vi "Query Mast Position.vi"(8 "error in (no error)":errorcluster, 11 "CO3000 in":refnum<class "CO3000.lvclass">) -> (0 "error out":errorcluster, 2 "Current Position (in cm)":i32, 3 "CO3000 out":refnum<class "CO3000.lvclass">)   [LabVIEW 2023, in "Turn Table and Mast.lvlib" / "CO3000.lvclass"]
uses:
  CO3000.lvclass
  CO3000.lvclass/CO3000.ctl
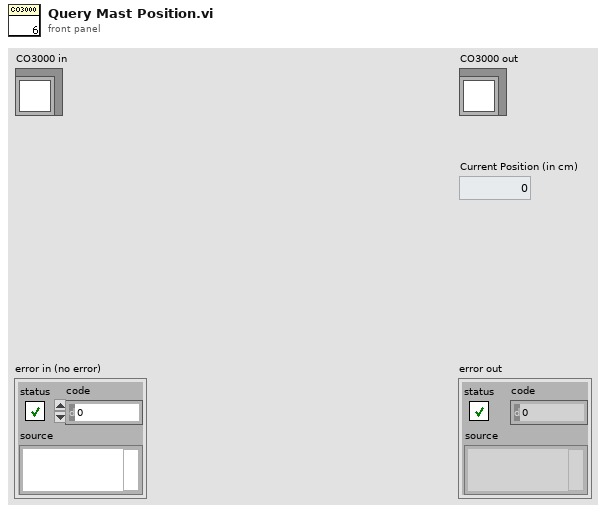
[diagram p1: front panel]
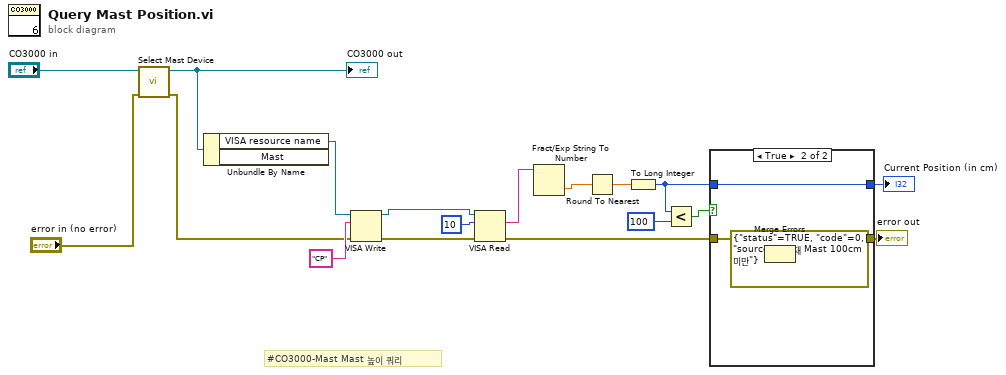
[diagram p0: block diagram]
diagram:
  # "#CO3000-Mast Mast 높이 쿼리"
  n1 = call "Select Mast Device.vi"("error in (no error)"="error in (no error)", "CO3000 in"="CO3000 in") -> ("error out"=w2:errorcluster, "CO3000 out"=w1:refnum<class "CO3000.lvclass">)  [unwired: 8 in]
  "CO3000 out" <- w1
  n2 = Unbundle By Name(w1) -> ("VISA resource name"=w14:refnum<visa-resource-name>)  [unwired: 1 out]
  n3 = VISA Write(VISA resource name=w14, write buffer="CP" ("버퍼 쓰기"), error in (no error)=w2) -> (VISA resource name out=w16:refnum<visa-resource-name>, error out=w17:errorcluster)  [unwired: 1 out]
  n4 = VISA Read(VISA resource name=w16, byte count=u32 10 ("바이트 카운트"), error in (no error)=w17) -> (read buffer=w13:string, error out=w6:errorcluster)  [unwired: 2 out]
  n5 = Fract/Exp String To Number(string=w13) -> (number=w12:dbl)  [unwired: 3 in, 1 out]
  n6 = Round To Nearest(number=w12) -> (nearest integer value=w11:dbl)
  n7 = To Long Integer(number=w11) -> (32bit integer=w8:i32)
  n8 = Less?(x=w8, y=100) -> (x < y?=w9:bool)
  n9 = case shown="True" w9 {
    tunnel: w8 -> [w20 w24]
    tunnel: [w20 w24] -> w7
    tunnel: w6 -> [w19 w22]
    tunnel: [w19 w21] -> w5
    frame False {
    }
    frame True {
      n10 = Merge Errors(w22, errorcluster {"status"=TRUE, "code"=0, "source"="현재 Mast 100cm 미만"} ("error out")) -> (w21:errorcluster)
    }
  }
  "error out" <- w5
  "Current Position (in cm)" <- w7
